vi "Verify Bitfile Versions Can Support Additional Bitfile.vi"(8 "error in (no error)":errorcluster, 10 "RIO Device Addresses":string[](array[string]), 11 "Item Ref in":T1 format="%.0x") -> (0 "error out":errorcluster, 2 "Can Add?":bool, 3 "Item Ref out":T1 format="%.0x")   [LabVIEW 2020, in "Engine Simulation Toolkit System Explorer.lvlib"]
uses:
  Engine Simulation Toolkit System Explorer.lvlib
  <vilib>/NI VeriStand/Custom Device API/Custom Device Item Ref.ctl
  Shared/Properties.vi
  Shared/Constants and GUIDs.vi
  <vilib>/NI VeriStand/Custom Device API/Get Item Property (String).vi
  Shared/Engine Simulation Toolkit Shared.lvlib
  <vilib>/NI VeriStand/Custom Device API/Custom Device API.lvlib
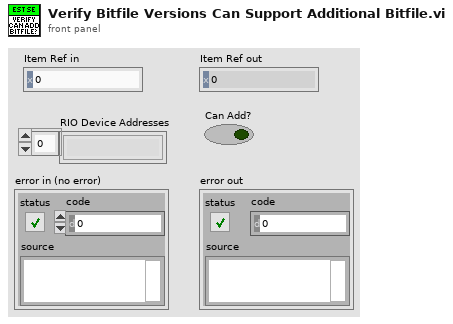
[diagram p1: front panel]
types:
  T1 = typedef "Custom Device API.lvlib/Custom Device Item Ref.ctl" = u64
  T2 = typedef "Engine Simulation Toolkit Shared.lvlib/Bitfile EST Version.ctl" = enum16{"1.0", "1.1", "1.2", "1.3", "1.4"}
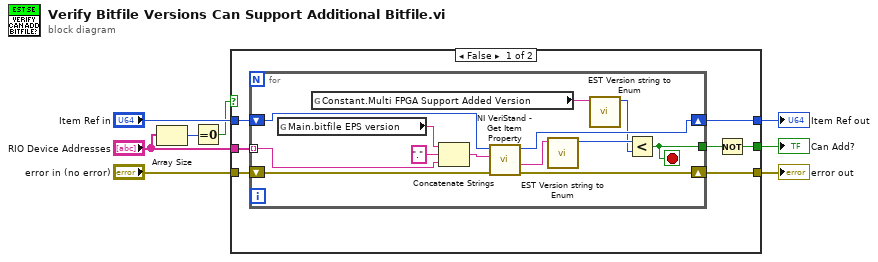
[diagram p0: block diagram]
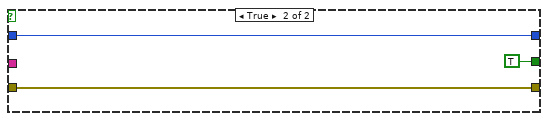
[diagram p2: hidden frame]
diagram:
  n1 = Array Size(array="RIO Device Addresses") -> (size(s)=w2:i32)
  n2 = Equal To 0?(x=w2) -> (x = 0?=w1:bool)
  n3 = case shown="False" w1 {
    tunnel: [w14 w29] -> w8
    tunnel: "Item Ref in" -> [w13 w29]
    tunnel: [w12 w30] -> w6
    tunnel: "error in (no error)" -> [w11 w30]
    tunnel: [w10 TRUE] -> w4
    tunnel: "RIO Device Addresses" -> [w9 _]
    frame False {
      n4 = for {
        tunnel: w9 -> [w26] mode=indexing
        shift-right: [w24] -> w12
        shift-left: w11 -> [w25]
        shift-right: [w21] -> w14
        shift-left: w13 -> [w22]
        tunnel: [w18] -> w15
        stop <- w18 stop-if-true
        n5 = global read "Properties.vi" "Main.bitfile EPS version"() -> (w28:string)
        n6 = global read "Constants and GUIDs.vi" "Constant.Multi FPGA Support Added Version"() -> (w17:string)
        n7 = Concatenate Strings(w28, "." ("string"), w26) -> (w23:string)
        n8 = call-poly <vilib>:"NI VeriStand - Get Item Property.vi"("error in (no error)"=w25, "Property Name"=w23, "Item Ref in"=w22) -> ("error out"=w24:errorcluster, "Value"=w20:string, "Item Ref out"=w21:T1)  [unwired: 5 in, 1 out]
        n9 = call "EST Version string to Enum.vi"("EST version string"=w20) -> ("EST version enum"=w19:T2)  [unwired: 9 in, 1 out]
        n10 = call "EST Version string to Enum.vi"("EST version string"=w17) -> ("EST version enum"=w16:T2)  [unwired: 9 in, 1 out]
        n11 = Less?(x=w19, y=w16) -> (x < y?=w18:bool)
      }
      n12 = Not(x=w15) -> (.not. x?=w10:bool)
    }
    frame True {
    }
  }
  "Can Add?" <- w4
  "Item Ref out" <- w8
  "error out" <- w6
